vi "Logging.vi"(7 "CSM Name":string="CSM-Module") -> ()   [LabVIEW 2026, in "UI-无创.lvlib" / "Logging.lvlib"]
uses:
  Logging.lvlib
  Supports/Logging States.ctl
  Supports/Sample Settings.ctl
  Supports/Time and Data_OP.ctl
  4d3beaf1-401a-43cb-9e41-e4ff7a78e202.vi
  1a146c5b-3d51-4d3e-9388-f96b0b9a5a8e.vi
  <userlib>/_NEVSTOP/Communicable State Machine(CSM)/AdvanceAPI/CSM - Revert Arguments-Safe String.vi
  <userlib>/_NEVSTOP/Communicable State Machine(CSM)/_Shared/Trim Single-line Text.vi
  <userlib>/_NEVSTOP/Communicable State Machine(CSM)/AdvanceAPI/CSM - Make String Arguments Safe.vi
  <userlib>/_NEVSTOP/Communicable State Machine(CSM)/AdvanceAPI/CSM - Break Down Multiple States String.vi
  <userlib>/_NEVSTOP/Communicable State Machine(CSM)/AdvanceAPI/CSM - Compact Multiple States.vi
  <userlib>/_NEVSTOP/Communicable State Machine(CSM)/AdvanceAPI/CSM - Keywords.vi
  <userlib>/_NEVSTOP/Communicable State Machine(CSM)/addons/API-String-Arugments-Support/_Support/Convert API String Arguments to Data(variant).vi
  <userlib>/_NEVSTOP/Communicable State Machine(CSM)/addons/MassData-Parameter/_support/FGV-MassData(lvlibp).vi
  <userlib>/_NEVSTOP/Communicable State Machine(CSM)/Communicable State Machine.lvlib
panel:
  out "Error Occurred":errorcluster
  out "State History":string
  in  "Exit":bool
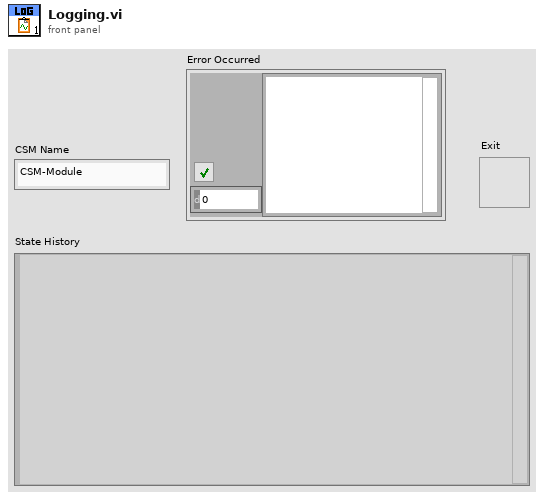
[diagram p1: front panel]
types:
  T1 = enum32{"Invalid", "Standard", "Closed", "Hidden", "Minimized", "Maximized"}
  T2 = enum32{"invalid app kind", "Development System", "Run Time System", "Student Edition", "Embedded LabVIEW", "Evaluation", "Custom"}
  T3 = typedef "UI-无创.lvlib/Logging.lvlib/Logging States.ctl" = enum16{"Idle", "Logging", "Error"}
  T4 = typedef "Communicable State Machine.lvlib/_CSM_Response Source Message.ctl" = cluster{"‘State":string, "’Arguments":string, "’Error":errorcluster}
  T5 = cluster{"Current VI Reference":refnum<vi>, "Close Panel on Exit?":bool}
  T6 = typedef "UI-无创.lvlib/Sample Settings.ctl" = cluster{"设备信息":cluster{"初始索引子集":i8[], "模拟信号采集通道":string, "数字-供电":refnum<k21>, "数字-光控":refnum<k21>, "光控设备":tag, "光电设备分离？":bool, "光谱保存路径":path, "环数":u8}, "测量控制":cluster{"测头拿起":bool, "起始保存":bool, "测头供电":bool, "测头出光":bool}, "测量":cluster{"每波长测量次数":i32, "波长":i32[], "起始周期":i32, "起始测量周期":i32}, "等待":cluster{"等待时间(s)":dbl, "等待方式":bool, "每x周期/点等待":i32, "等待时":enum16{"无电无光", "有电无光", "无电有光", "有电有光"}}, "校准":cluster{"暗电流校准值初值":dbl[], "温度校准值":dbl[], "校准模式":T7}, "图表相关":cluster{"文件-时间":string}, "CSM":cluster{"CSM Name":string}}
  T7 = typedef "UI-无创.lvlib/暗电流校准模式.ctl" = enum32{"手动", "逐周期"}
  T8 = cluster{"Core":cluster{"Current VI Reference":refnum<vi>, "Close Panel on Exit?":bool}, "Logging State":T3, "Sample Settings":T6}
  T9 = typedef "UI-无创.lvlib/Time and Data_OP.ctl" = cluster{"采集时间":timestamp, "采集时间(dbl)":dbl, "Data":dbl[], "当前运行信息":cluster{"当前周期":i32, "当前次数":i32, "测量周期":i32, "当前索引子集":i8[], "当前波长":i32}, "暗电流校准值":dbl[], "Logging Settings":cluster{"是否保存？":bool, "波长结束？":bool, "周期结束？":bool}, "原始值":cluster{"1环(原始值)":dbl[][], "2环(原始值)":dbl[][], "3环(原始值)":dbl[][], "4环(原始值)":dbl[][], "5环(原始值)":dbl[][], "6环(原始值)":dbl[][], "7环(原始值)":dbl[][]}, "校准值":cluster{"1环(校准值)":dbl[][], "2环(校准值)":dbl[][], "3环(校准值)":dbl[][], "4环(校准值)":dbl[][], "5环(校准值)":dbl[][], "6环(校准值)":dbl[][], "7环(校准值)":dbl[][]}}
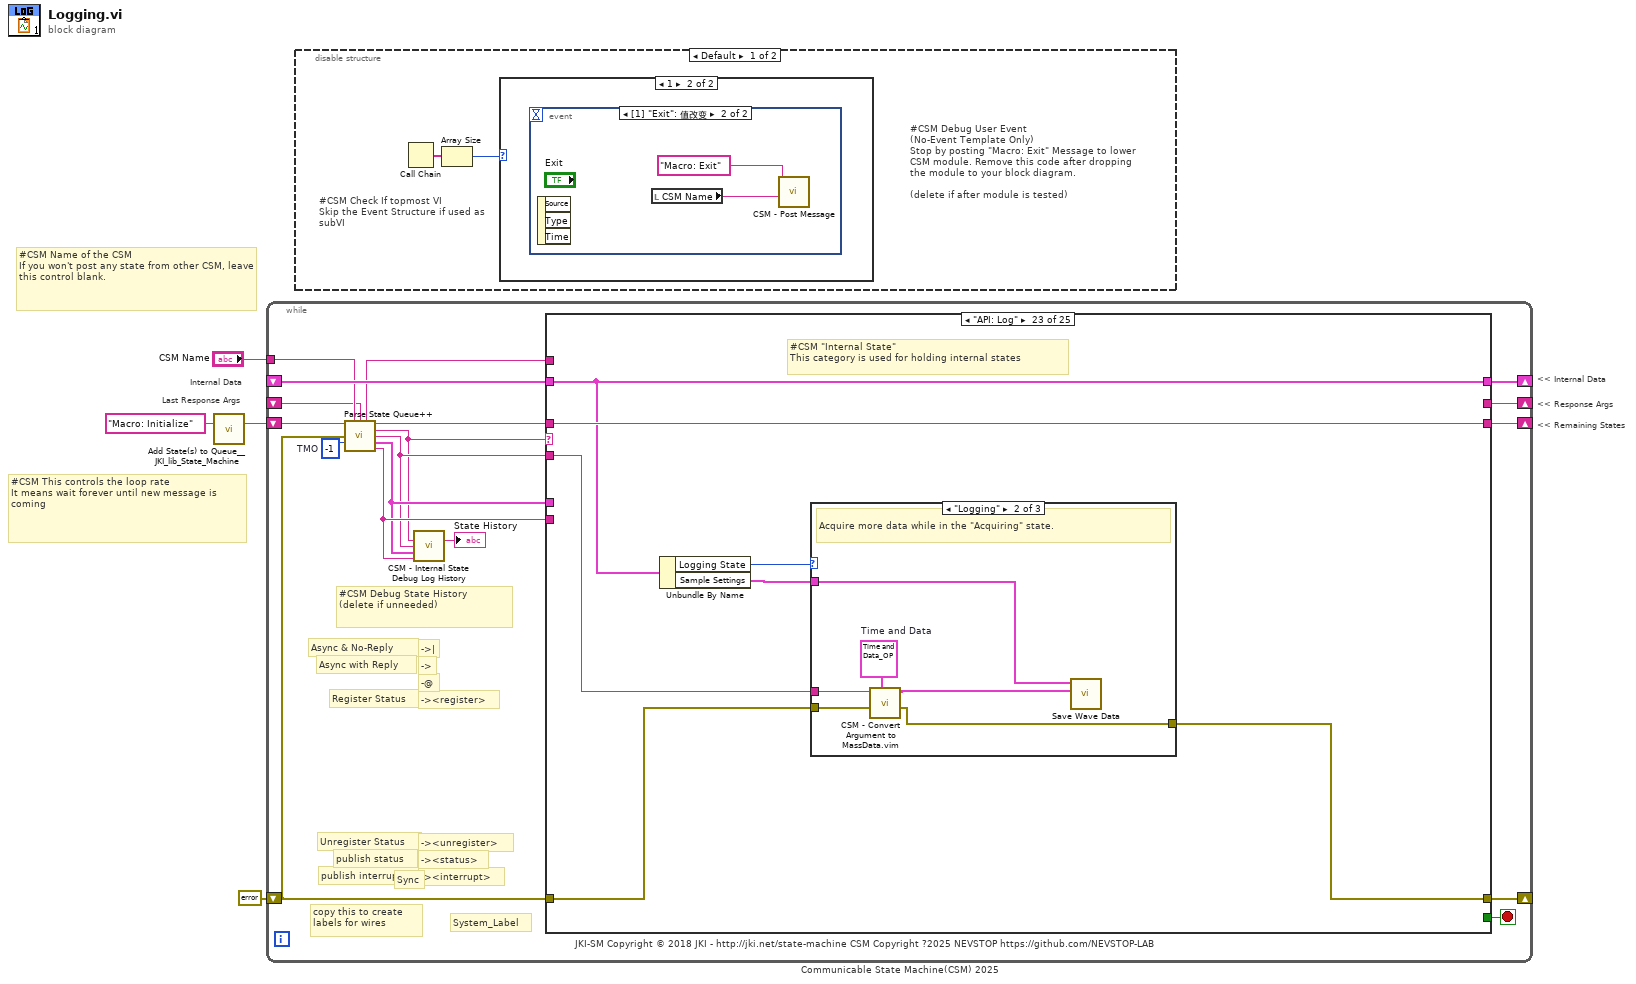
[diagram p0: block diagram]
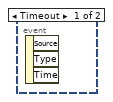
[diagram p3: hidden frame]
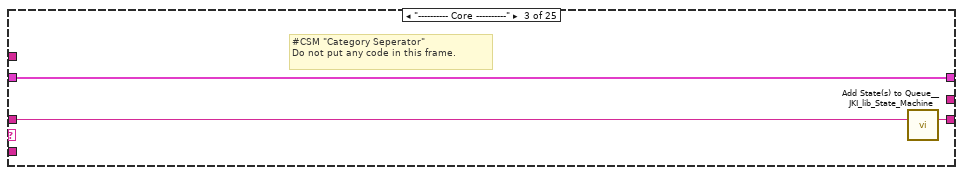
[diagram p7: hidden frame]
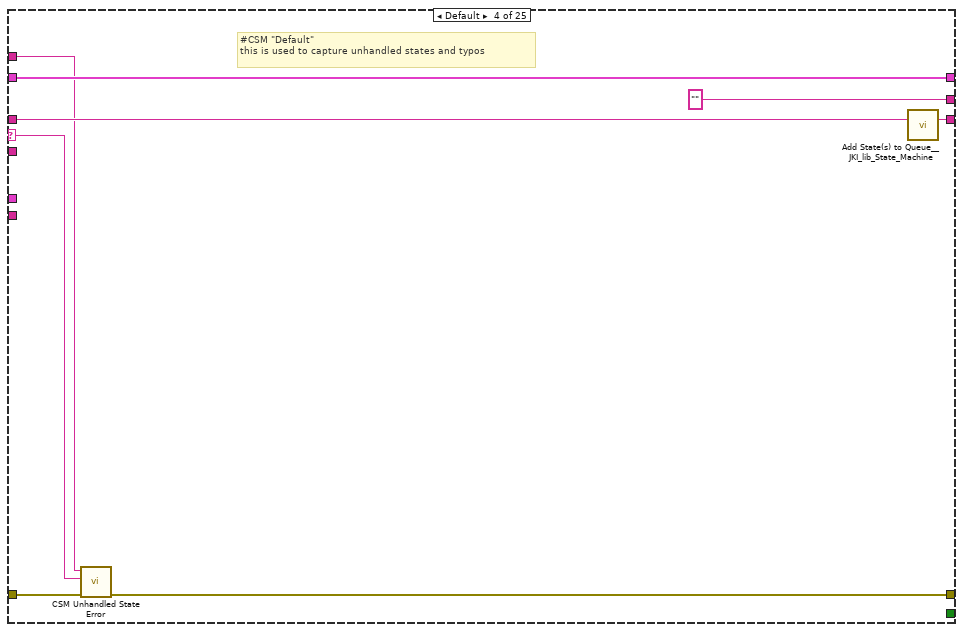
[diagram p8: hidden frame]
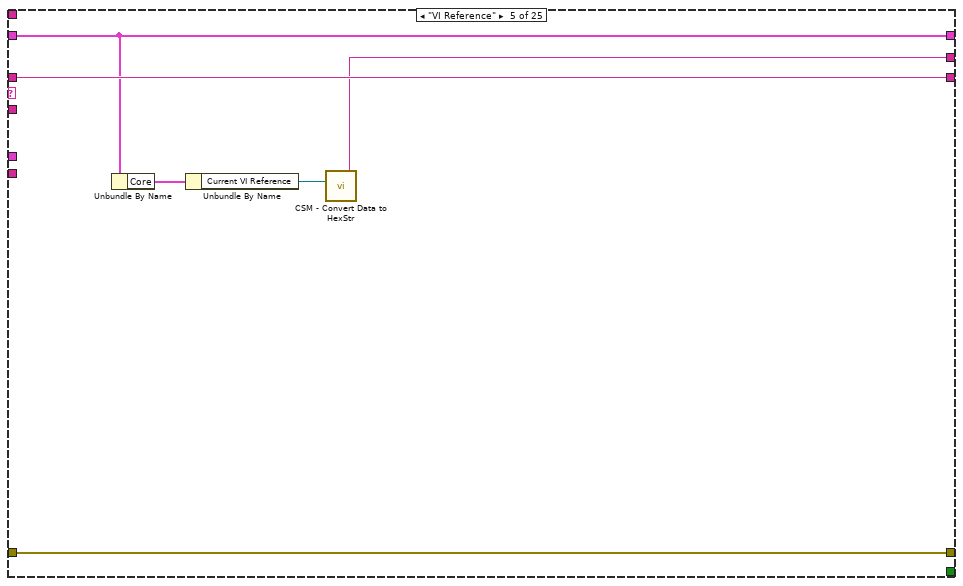
[diagram p9: hidden frame]
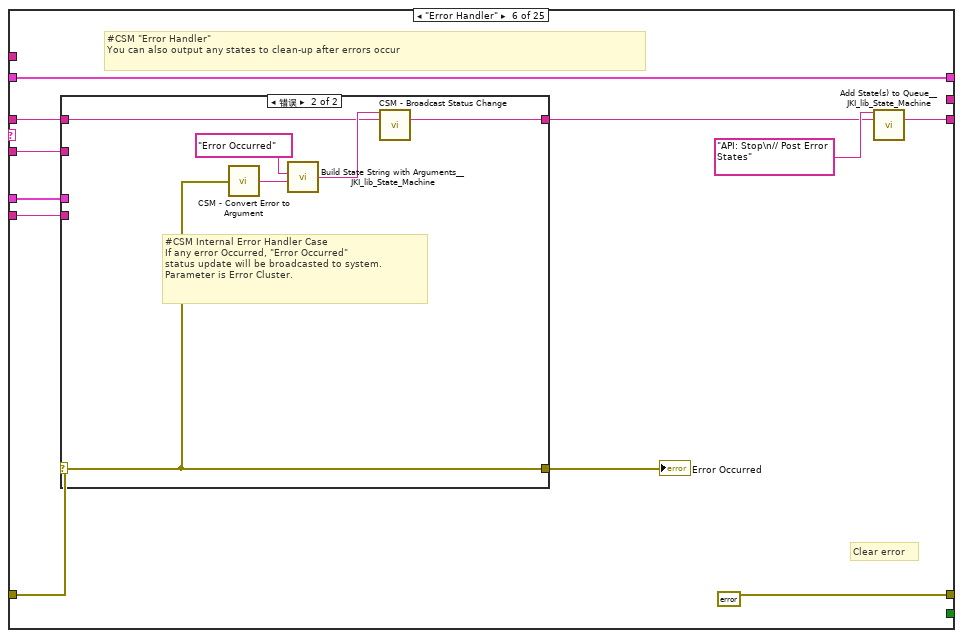
[diagram p10: hidden frame]
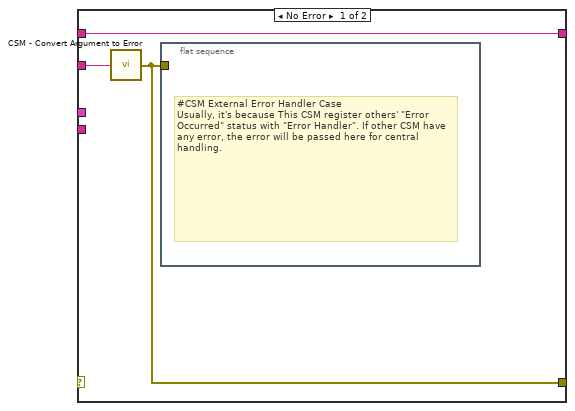
[diagram p11: hidden frame]
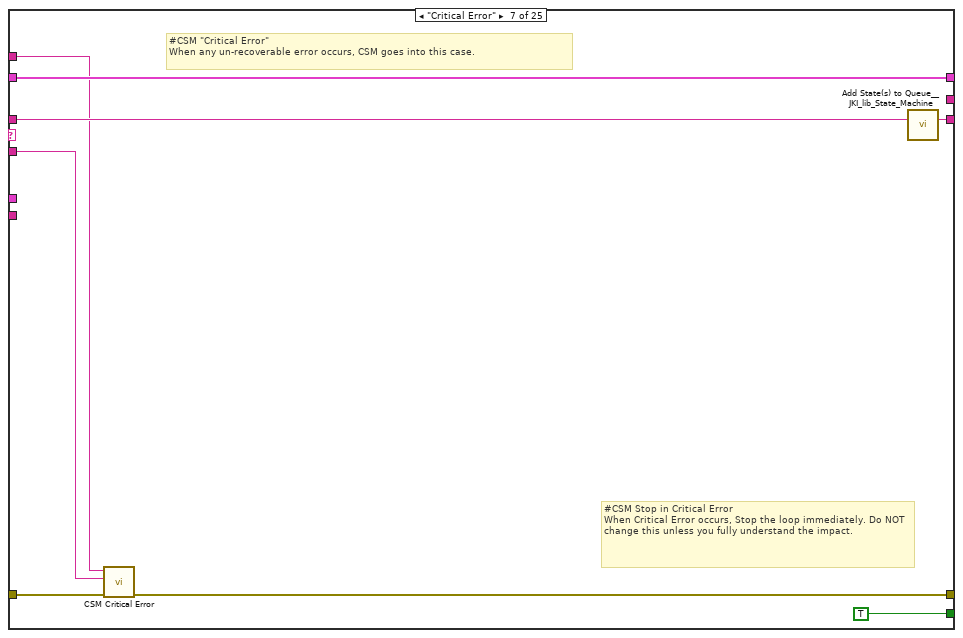
[diagram p12: hidden frame]
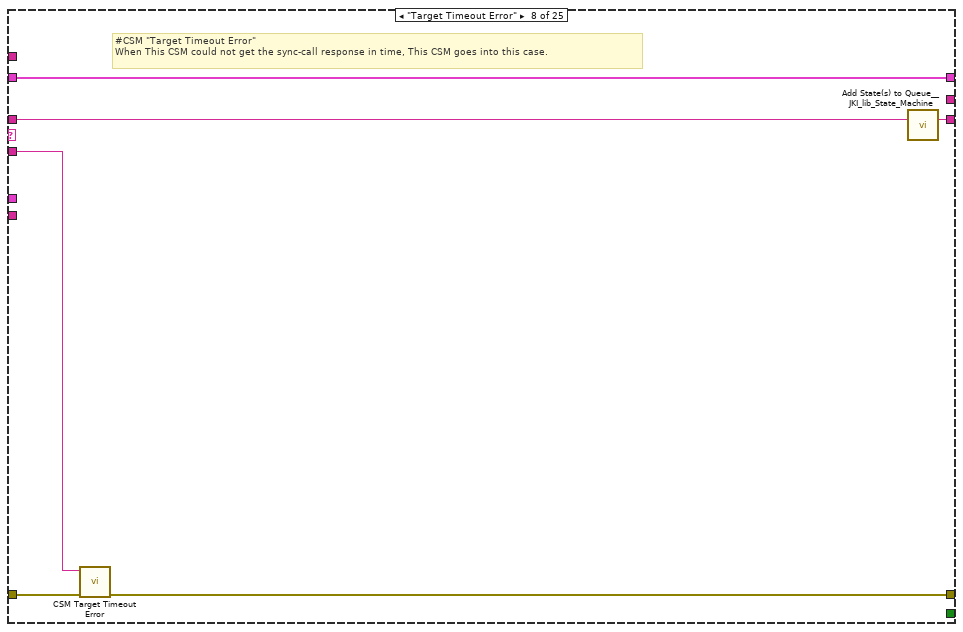
[diagram p13: hidden frame]
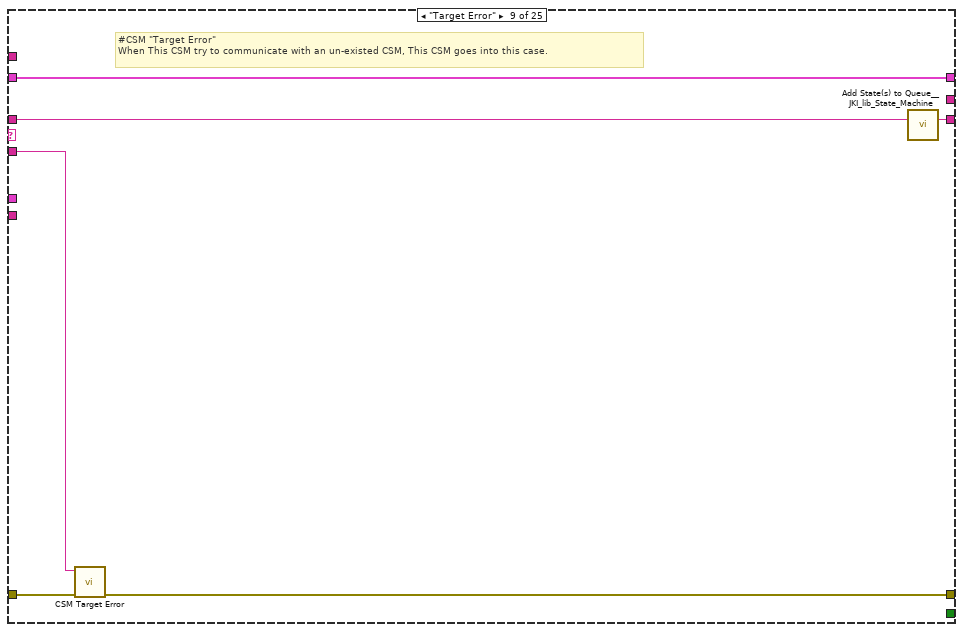
[diagram p14: hidden frame]
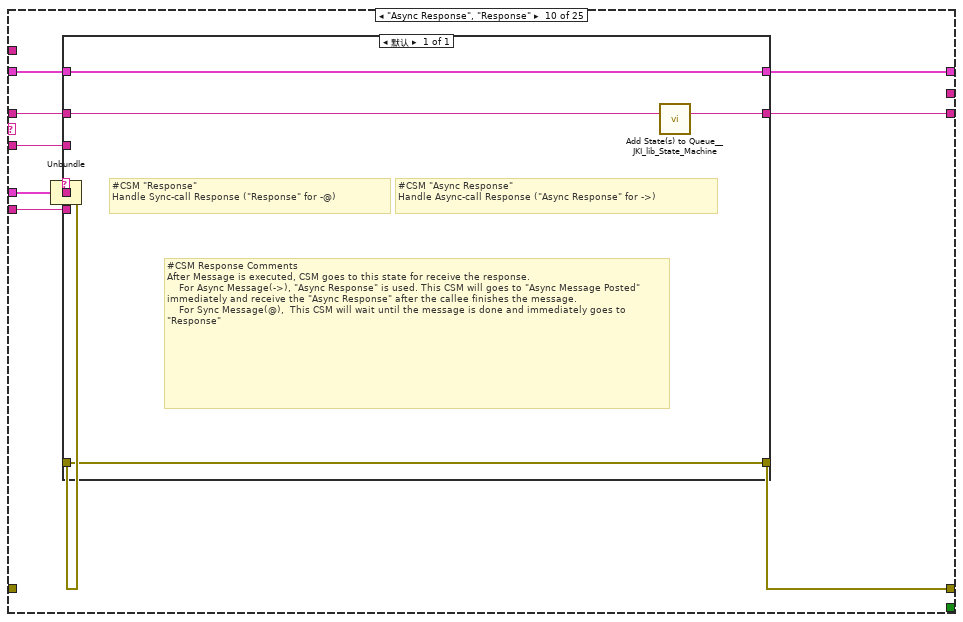
[diagram p15: hidden frame]
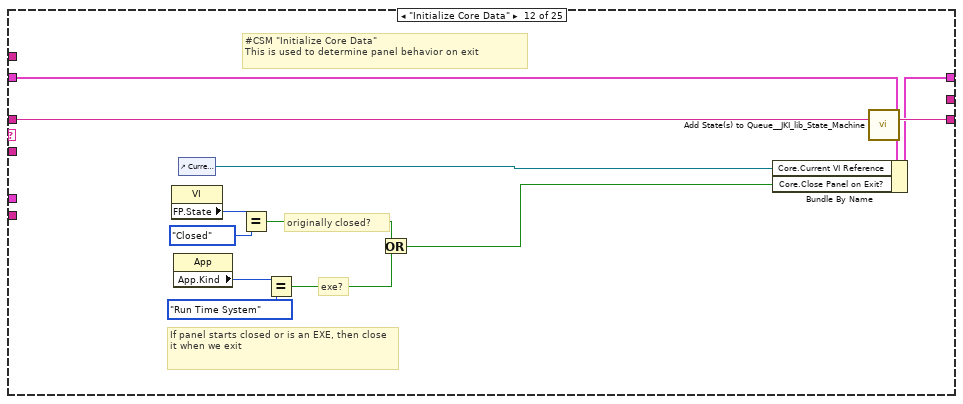
[diagram p17: hidden frame]
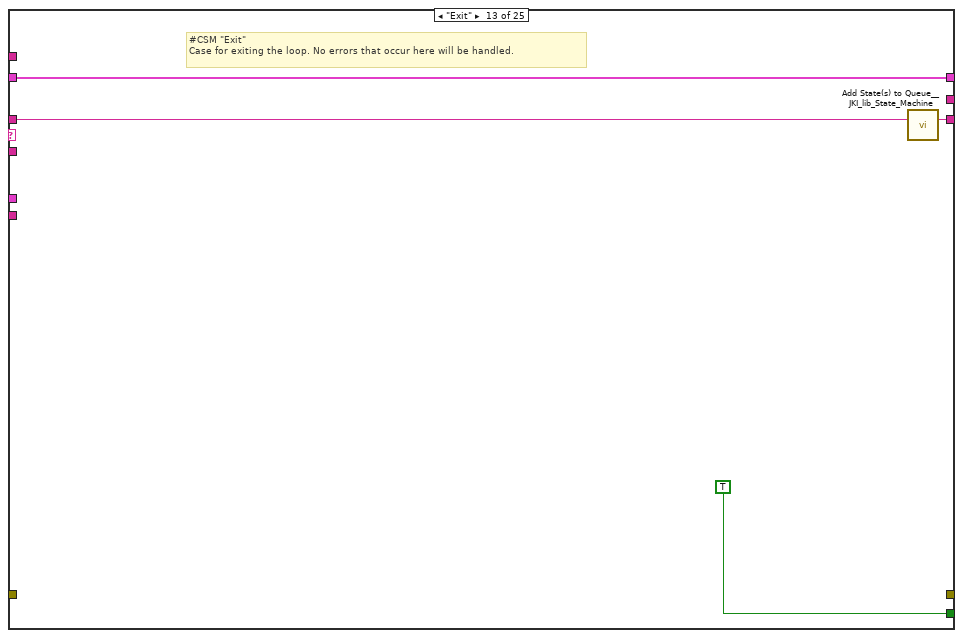
[diagram p18: hidden frame]
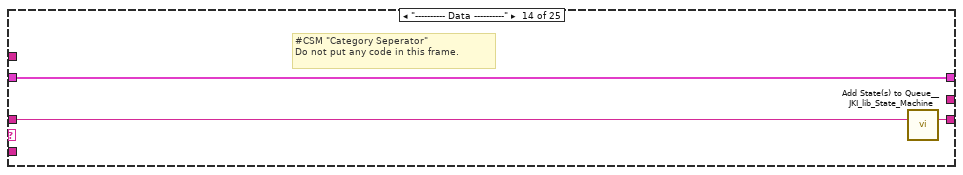
[diagram p19: hidden frame]
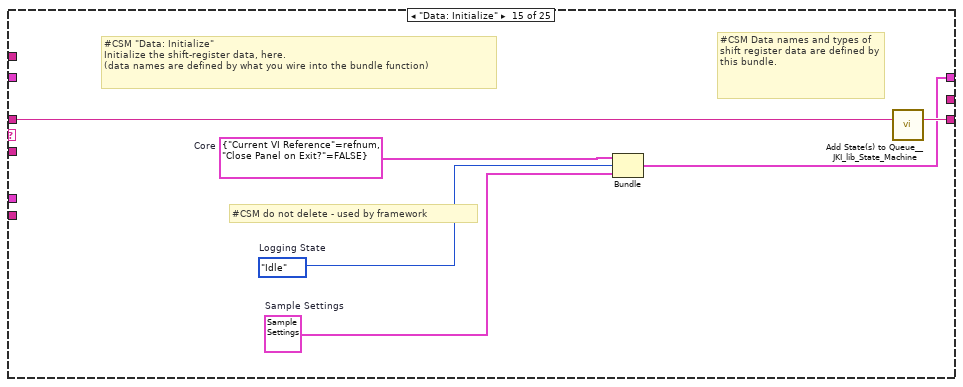
[diagram p20: hidden frame]
diagram:
  # "Last Response Args"
  # "Internal Data"
  # "#CSM Name of the CSM\nIf you won't post any state from other CSM, leave this control blank."
  # "#CSM This controls the loop rate\nIt means wait forever until new message is coming"
  # "<< Internal Data"
  # "<< Response Args"
  # "<< Remaining States"
  n1 = call <vilib>:"Add State(s) to Queue__JKI_lib_State_Machine.vi"("State(s) in (\"\")"="Macro: Initialize" ("Init State(\"Macro: Initialize\")")) -> ("States Out"=w1:string)  [unwired: 14 in]
  n2 = while "Communicable State Machine(CSM) 2025" {
    shift-right: [w17] -> _
    shift-left: _ -> [w16]
    shift-right: [w20] -> _
    shift-left: errorcluster {"status"=FALSE, "code"=0, "source"=""} ("error out") -> [w6]
    shift-right: [w19] -> _
    shift-left: w1 -> [w21]
    tunnel: "CSM Name" -> [w13]
    shift-right: [w14] -> _
    shift-left: _ -> [w8]
    stop <- w18 stop-if-true
    w15 = -1  # TMO
    # "#CSM Debug State History\n(delete if unneeded)"
    # "-><interrupt>"
    # "-><status>"
    # "-><unregister>"
    # "-><register>"
    # "-@"
    # "->"
    # "->|"
    # "publish interrupt"
    # "publish status"
    # "Unregister Status"
    # "Register Status"
    # "Sync"
    # "Async with Reply"
    # "Async & No-Reply"
    # "JKI-SM Copyright © 2018 JKI - http://jki.net/state-machine CSM Copyright ?2025 NEVSTOP https://github.com/NEVSTOP-LAB"
    # "copy this to create labels for wires"
    # "System_Label"
    n3 = call <userlib>:"Parse State Queue++.vi"("State Queue"=w21, "Name (\"\" to Use UUID)"=w13, "Response Arguments"=w8, "Previous Error"=w6, "Dequeue (1 ms)"=w15) -> ("Name Used"=w7:string, "Remaining States"=w22:string, "Current State"=w9:string, "Arguments"=w10:string, "Additional Information"=w11:T4, "Source CSM"=w12:string)  [unwired: 5 in]
    n4 = call <userlib>:"CSM - Internal State Debug Log History.vi"("State"=w9, "Arguments (\"\")"=w10, ">> Response Source Message >>"=w11, "Source (\"\")"=w12) -> ("Debug Log"=→"State History":string)  [unwired: 11 in]
    n5 = case shown="\"API: Log\"" w9 {
      selector: w9 -> [_ _ _ w33 _ _ _ _ _ _ _ _ _ _ _ _ _ _ _ _ _ _ _ _ _]
      tunnel: w22 -> [w23 w26 w29 w37 w42 w48 w71 w77 w83 w93 w100 w112 w116 w119 w125 w128 w134 w137 w141 w147 w149 w156 w170 w184 w193]
      tunnel: w10 -> [_ _ _ _ _ w47 w67 w74 w80 w87 _ _ _ _ _ _ _ _ _ _ _ w151 w168 _ _]
      tunnel: w16 -> [w24 w25 w27 w35 w41 w53 w69 w75 w81 w91 w99 w106 w114 w117 _ w127 w129 w135 w139 w145 w150 w155 w169 w185 w191]
      tunnel: [_ _ _ w30 w43 errorcluster {"status"=FALSE, "code"=0, "source"=""} ("error out") w64 w72 w78 w94 _ _ _ _ _ _ w130 _ _ _ _ w152 w171 _ _] -> w20
      tunnel: w6 -> [_ _ _ w31 w43 w51 w65 w73 w79 _ _ _ _ _ _ _ w131 _ _ _ _ w152 w172 _ _]
      tunnel: [w23 w26 w28 w36 w42 w49 w70 w76 w82 w92 w100 w111 w115 w118 w124 w128 w133 w136 w140 w146 w148 w156 w170 w183 w192] -> w19
      tunnel: [_ _ _ _ _ _ TRUE _ _ _ _ _ TRUE _ _ _ _ _ _ _ _ _ _ _ _] -> w18
      tunnel: [w24 w25 w27 w35 w41 w53 w69 w75 w81 w90 w99 w110 w114 w117 w123 w127 w129 w135 w139 w145 w150 w154 w169 w185 w190] -> w17
      tunnel: w12 -> [_ _ _ _ _ w46 _ _ _ w88 _ _ _ _ _ _ _ _ _ _ _ _ _ _ _]
      tunnel: w11 -> [_ _ _ _ _ w45 _ _ _ w89 _ _ _ _ _ _ _ _ _ _ _ _ _ _ _]
      tunnel: [_ _ _ "" w38 _ _ _ _ _ _ _ _ _ _ _ _ _ _ _ _ _ _ _ _] -> w14
      tunnel: w7 -> [_ _ _ w32 _ _ w66 _ _ _ _ _ _ _ _ _ _ _ _ _ _ w153 _ _ _]
      frame "", "Idle" {
        # "#CSM \"Idle/Event Handler\"\nexecutes when the state queue is empty"
      }
      frame "CSM Documentation" {
        # "#CSM State Syntax\n\n// Comment line, all text to the right of “//” will be ignored\n// Local Message Example\nDoSth: DoA >> Arguments\n\n// Sync Call Example\nAPI: xxxx >> Arguments -@ TargetModule\n\n// Async Call Example\nAPI: xxxx >> Arguments -> TargetModule\n\n// Async Call without Reply Example\nAPI: xxxx >> Arguments ->| TargetModule\n\n// Broadcast normal status:\nStatus >> StatusArguments  -><status>\n\n// Broadcast Interrupt status:\nInterrupt >> StatusArguments  -><interrupt>\n\n// Register Source Module's status to Handler Module\nStatus@Source Module >> Handler Module@Handler Module -><register>\n\n// Unegister Source Module's status\nStatus@Source Module >> Handler Module -><unregister>"
        # "#CSM README FIRST\n\nCommunicable State Machine(CSM) is a LabVIEW application framework that builds upon JKI State Machine(JKISM). It follows the pattern of JKISM and extends the keywords to describe message communication between modules, including concepts such as Sync-Message, Async-Message, Subscription/Unsubscription of status - essential elements for creating reusable code modules. For more information, please visit the CSM wiki: https://nevstop-lab.github.io/CSM-Wiki/\n\nFor instructions on JKI State Machine, visit: \n    http://jki.net/state-machine/\nFor information about CSM, visit: \n    https://github.com/NEVSTOP-LAB"
        # "#CSM \"Documentation\"\nCase for holding CSM Documenation"
      }
      frame "---------- Core ----------" {
        # "#CSM \"Category Seperator\"\nDo not put any code in this frame."
        n6 = call <vilib>:"Add State(s) to Queue__JKI_lib_State_Machine.vi"("State(s) in (\"\")"=w29) -> ("States Out"=w28:string)  [unwired: 14 in]
      }
      frame Default {
        # "#CSM \"Default\"\nthis is used to capture unhandled states and typos"
        n7 = call <userlib>:"CSM Unhandled State Error.vi"("error in (no error)"=w31, "Undefined State"=w33, "CSM Name"=w32) -> ("error out"=w30:errorcluster)  [unwired: 8 in]
        n8 = call <vilib>:"Add State(s) to Queue__JKI_lib_State_Machine.vi"("State(s) in (\"\")"=w37) -> ("States Out"=w36:string)  [unwired: 14 in]
      }
      frame "VI Reference" {
        n9 = Unbundle By Name(w41) -> ("Core"=w40:T5)
        n10 = Unbundle By Name(w40) -> ("Current VI Reference"=w39:refnum<vi>)
        n11 = call <userlib>:"CSM - Convert Data to HexStr.vi"("Variant"=w39) -> ("HEX String (0-9,A-F)"=w38:string)  [unwired: 8 in]
      }
      frame "Error Handler" {
        # "#CSM \"Error Handler\"\nYou can also output any states to clean-up after errors occur"
        # "Clear error"
        n12 = case shown="错误" w51 {
          selector: w51 -> [_ w58]
          tunnel: [w57 w60] -> w50
          tunnel: w48 -> [w57 w59]
          tunnel: w47 -> [w56 _]
          tunnel: w46 -> [_ _]
          tunnel: w45 -> [_ _]
          tunnel: [w55 w58] -> w44
          frame No Error {
            n13 = call <userlib>:"CSM - Convert Argument to Error.vi"("Argument"=w56) -> ("Error"=w55:errorcluster)  [unwired: 4 in]
            n14 = flat-sequence {
              tunnel: w55 -> [_]
              frame #0 {
                # "#CSM External Error Handler Case\nUsually, it's because This CSM register others' \"Error Occurred\" status with \"Error Handler\". If other CSM have any error, the error will be passed here for central handling."
              }
            }
          }
          frame Error {
            # "#CSM Internal Error Handler Case \nIf any error Occurred, \"Error Occurred\" \nstatus update will be broadcasted to system.\nParameter is Error Cluster."
            n15 = call <userlib>:"CSM - Convert Error to Argument.vi"("Error"=w58) -> ("Argument"=w62:string)  [unwired: 4 in]
            n16 = call <vilib>:"Build State String with Arguments__JKI_lib_State_Machine.vi"("Arguments (\"\")"=w62, "State"="Error Occurred" ("Status with Arguments")) -> ("State with Arguments"=w61:string)  [unwired: 4 in]
            n17 = call <userlib>:"CSM - Broadcast Status Change.vi"("Status With Arguments"=w61, "State Queue"=w59) -> ("Remaining States"=w60:string)  [unwired: 13 in]
          }
        }
        "Error Occurred" <- w44
        n18 = call <vilib>:"Add State(s) to Queue__JKI_lib_State_Machine.vi"("State(s) in Front (\"\")"="API: Stop\n// Post Error States", "State(s) in (\"\")"=w50) -> ("States Out"=w49:string)  [unwired: 13 in]
      }
      frame "Critical Error" {
        # "#CSM \"Critical Error\"\nWhen any un-recoverable error occurs, CSM goes into this case."
        # "#CSM Stop in Critical Error\nWhen Critical Error occurs, Stop the loop immediately. Do NOT change this unless you fully understand the impact."
        n19 = call <userlib>:"CSM Critical Error.vi"("error in (no error)"=w65, "Arugments (As Reason)"=w67, "CSM Name"=w66) -> ("error out"=w64:errorcluster)  [unwired: 8 in]
        n20 = call <vilib>:"Add State(s) to Queue__JKI_lib_State_Machine.vi"("State(s) in (\"\")"=w71) -> ("States Out"=w70:string)  [unwired: 14 in]
      }
      frame "Target Timeout Error" {
        # "#CSM \"Target Timeout Error\"\nWhen This CSM could not get the sync-call response in time, This CSM goes into this case."
        n21 = call <userlib>:"CSM Target Timeout Error.vi"("error in (no error)"=w73, "Arguments (As CSM Name)"=w74) -> ("error out"=w72:errorcluster)  [unwired: 9 in]
        n22 = call <vilib>:"Add State(s) to Queue__JKI_lib_State_Machine.vi"("State(s) in (\"\")"=w77) -> ("States Out"=w76:string)  [unwired: 14 in]
      }
      frame "Target Error" {
        # "#CSM \"Target Error\"\nWhen This CSM try to communicate with an un-existed CSM, This CSM goes into this case."
        n23 = call <userlib>:"CSM Target Error.vi"("error in (no error)"=w79, "Arguments (As CSM Name)"=w80) -> ("error out"=w78:errorcluster)  [unwired: 9 in]
        n24 = call <vilib>:"Add State(s) to Queue__JKI_lib_State_Machine.vi"("State(s) in (\"\")"=w83) -> ("States Out"=w82:string)  [unwired: 14 in]
      }
      frame "Async Response", "Response" {
        n25 = Unbundle(w89) -> ("‘State"=w86:string, "’Arguments"=w85:string, "’Error"=w84:errorcluster)
        n26 = case shown="默认" w86 {
          tunnel: [w95] -> w92
          tunnel: w93 -> [w96]
          tunnel: [w98] -> w90
          tunnel: w91 -> [w98]
          tunnel: [w97] -> w94
          tunnel: w84 -> [w97]
          tunnel: w88 -> [_]
          tunnel: w87 -> [_]
          tunnel: w85 -> [_]
          frame 默认 {
            # "#CSM \"Async Response\"\nHandle Async-call Response (\"Async Response\" for ->)"
            # "#CSM \"Response\"\nHandle Sync-call Response (\"Response\" for -@)"
            # "#CSM Response Comments\nAfter Message is executed, CSM goes to this state for receive the response.\n    For Async Message(->), \"Async Response\" is used. This CSM will goes to \"Async Message Posted\" immediately and receive the \"Async Response\" after the callee finishes the message.\n    For Sync Message(@),  This CSM will wait until the message is done and immediately goes to \"Response\""
            n27 = call <vilib>:"Add State(s) to Queue__JKI_lib_State_Machine.vi"("State(s) in (\"\")"=w96) -> ("States Out"=w95:string)  [unwired: 14 in]
          }
        }
      }
      frame "Async Message Posted" {
        # "#CSM \"Async Message Posted\"\nAfter Async Message is posted (-> or ->| ), CSM goes to this state for post-action.\nYou can use Argument - State to tell which Async Message is called."
      }
      frame "Initialize Core Data" {
        # "#CSM \"Initialize Core Data\"\nThis is used to determine panel behavior on exit"
        # "originally closed?"
        # "exe?"
        # "If panel starts closed or is an EXE, then close it when we exit"
        n28 = property class="VI"() -> ("FP.State"=w103:T1)  [unwired: 2 in, 2 out]
        n29 = property class="App"() -> ("App.Kind"=w109:T2)  [unwired: 2 in, 2 out]
        n30 = control-ref of="Current VI Reference"() -> (w104:refnum<vi>)
        n31 = Equal?(x=w103, y=T1."Closed" ("Front Panel Window:State")) -> (x = y?=w101:bool)
        n32 = Equal?(x=w109, y=T2."Run Time System" ("Application:Kind")) -> (x = y?=w107:bool)
        n33 = Or(x=w101, y=w107) -> (x .or. y?=w105:bool)
        n34 = Bundle By Name(cluster=w106, "Core.Current VI Reference"=w104, "Core.Close Panel on Exit?"=w105) -> (w110:T8)
        n35 = call <vilib>:"Add State(s) to Queue__JKI_lib_State_Machine.vi"("State(s) in (\"\")"=w112) -> ("States Out"=w111:string)  [unwired: 14 in]
      }
      frame "Exit" {
        # "#CSM \"Exit\"\nCase for exiting the loop. No errors that occur here will be handled."
        n36 = call <vilib>:"Add State(s) to Queue__JKI_lib_State_Machine.vi"("State(s) in (\"\")"=w116) -> ("States Out"=w115:string)  [unwired: 14 in]
      }
      frame "---------- Data ----------" {
        # "#CSM \"Category Seperator\"\nDo not put any code in this frame."
        n37 = call <vilib>:"Add State(s) to Queue__JKI_lib_State_Machine.vi"("State(s) in (\"\")"=w119) -> ("States Out"=w118:string)  [unwired: 14 in]
      }
      frame "Data: Initialize" {
        w120 = T6 {"设备信息"={"初始索引子集"=[], "模拟信号采集通道"="", "数字-供电"="", "数字-光控"="", "光控设备"="", "光电设备分离？"=FALSE, "光谱保存路径"=path "", "环数"=0}, "测量控制"={"测头拿起"=FALSE, "起始保存"=FALSE, "测头供电"=TRUE, "测头出光"=TRUE}, "测量"={"每波长测量次数"=5, "波长"=[0, 0, 0, 0, 0, 0], "起始周期"=0, "起始测量周期"=0}, "等待"={"等待时间(s)"=0.0, "等待方式"=FALSE, "每x周期/点等待"=8, "等待时"=enum."无电无光"}, "校准"={"暗电流校准值初值"=[], "温度校准值"=[0.0, 0.0, 0.0, 0.0, 0.0, 0.0, 0.00013, 0.00013, 0.00013, 0.00013, 0.00013, 0.00013], "校准模式"=enum."逐周期"}, "图表相关"={"文件-时间"=""}, "CSM"={"CSM Name"=""}}  # Sample Settings
        w121 = Logging_States."Idle"  # Logging State
        w122 = T5 {"Current VI Reference"=refnum, "Close Panel on Exit?"=FALSE}  # Core
        # "#CSM \"Data: Initialize\"\nInitialize the shift-register data, here.\n(data names are defined by what you wire into the bundle function)"
        # "#CSM do not delete - used by framework"
        # "#CSM Data names and types of shift register data are defined by this bundle."
        n38 = Bundle("Core"=w122, "Logging State"=w121, "Sample Settings"=w120) -> (w123:T8)  [unwired: 1 in]
        n39 = call <vilib>:"Add State(s) to Queue__JKI_lib_State_Machine.vi"("State(s) in (\"\")"=w125) -> ("States Out"=w124:string)  [unwired: 14 in]
      }
      frame "Data: Update Indicators" {
        n40 = local write "Error Occurred"(errorcluster {"status"=FALSE, "code"=0, "source"=""} ("错误常量")) -> ()
      }
      frame "Data: Cleanup" {
        # "#CSM \"Data: Cleanup\"\nCleanup any data and references, here.\n(this is called automatically, by the Macro: Exit)"
        n41 = Unbundle By Name(w129) -> ("Core.Current VI Reference"=w132:refnum<vi>)
        n42 = Close Reference(reference=w132, error in (no error)=w131) -> (error out=w130:errorcluster)
        n43 = call <vilib>:"Add State(s) to Queue__JKI_lib_State_Machine.vi"("State(s) in (\"\")"=w134) -> ("States Out"=w133:string)  [unwired: 14 in]
      }
      frame "---------- Macro ----------" {
        # "#CSM \"Category Seperator\"\nDo not put any code in this frame."
        n44 = call <vilib>:"Add State(s) to Queue__JKI_lib_State_Machine.vi"("State(s) in (\"\")"=w137) -> ("States Out"=w136:string)  [unwired: 14 in]
      }
      frame "Macro: Initialize" {
        # "#CSM \"Macro: Initialize\"\nInitialization Macro (This is called once, when the VI starts)"
        n45 = call <vilib>:"Add State(s) to Queue__JKI_lib_State_Machine.vi"("State(s) in Front (\"\")"="Data: Initialize\nInitialize Core Data\nData: Update Indicators", "State(s) in (\"\")"=w141) -> ("States Out"=w140:string)  [unwired: 13 in]
      }
      frame "Macro: Exit" {
        # "#CSM \"Macro: Exit\"\nExit Macro (This is called once, when the VI exits)"
        n46 = call <vilib>:"Add State(s) to Queue__JKI_lib_State_Machine.vi"("State(s) in Front (\"\")"="//Exit Sub-Modules ", "State(s) at Back (\"\")"="Data: Cleanup\nExit") -> ("States Out"=w143:string)  [unwired: 13 in]
        n47 = call <vilib>:"Add State(s) to Queue__JKI_lib_State_Machine.vi"("State(s) in Front (\"\")"=w143, "State(s) in (\"\")"=w147) -> ("States Out"=w146:string)  [unwired: 13 in]
      }
      frame "---------- API ----------" {
        # "#CSM \"Category Seperator\"\nDo not put any code in this frame."
        n48 = call <vilib>:"Add State(s) to Queue__JKI_lib_State_Machine.vi"("State(s) in (\"\")"=w149) -> ("States Out"=w148:string)  [unwired: 14 in]
      }
      frame "API: Start" {
        # "#CSM API Example\nCopy/Rename this case for your own API"
        n49 = Unbundle By Name(w155) -> ("Logging State"=w158:T3)
        n50 = case shown="\"Idle\", 默认" w158 {
          tunnel: w155 -> [w164 w165 w166]
          tunnel: [w163 w165 w166] -> w154
          tunnel: w153 -> [_ _ _]
          tunnel: w151 -> [w161 _ _]
          frame "Idle", Default {
            w160 = T6 {"设备信息"={"初始索引子集"=[], "模拟信号采集通道"="", "数字-供电"="", "数字-光控"="", "光控设备"="", "光电设备分离？"=FALSE, "光谱保存路径"=path "", "环数"=0}, "测量控制"={"测头拿起"=FALSE, "起始保存"=FALSE, "测头供电"=TRUE, "测头出光"=TRUE}, "测量"={"每波长测量次数"=5, "波长"=[0, 0, 0, 0, 0, 0], "起始周期"=0, "起始测量周期"=0}, "等待"={"等待时间(s)"=0.0, "等待方式"=FALSE, "每x周期/点等待"=8, "等待时"=enum."无电无光"}, "校准"={"暗电流校准值初值"=[], "温度校准值"=[0.0, 0.0, 0.0, 0.0, 0.0, 0.0, 0.00013, 0.00013, 0.00013, 0.00013, 0.00013, 0.00013], "校准模式"=enum."逐周期"}, "图表相关"={"文件-时间"=""}, "CSM"={"CSM Name"=""}}  # Sample Settings
            # "If the system is idle, start the acquisition."
            n51 = call "Convert API String Arguments to Data.vim"("Reference Type"=w160, "API String"=w161) -> ("Data"=w159:T6)  [unwired: 6 in, 1 out]
            n52 = Bundle By Name(cluster=w164, "Logging State"=Logging_States."Logging", "Sample Settings"=w159) -> (w163:T8)
          }
          frame "Logging" {
            # "The system is already acquiring. Ignore the \"Start\" message."
          }
          frame "Error" {
          }
        }
        n53 = local write "Error Occurred"(errorcluster {"status"=FALSE, "code"=0, "source"=""} ("错误常量")) -> ()
      }
      frame "API: Log" {
        # "#CSM \"Internal State\"\nThis category is used for holding internal states"
        n54 = Unbundle By Name(w169) -> ("Logging State"=w173:T3, "Sample Settings"=w167:T6)
        n55 = case shown="\"Logging\"" w173 {
          tunnel: [w174 w177 w181] -> w171
          tunnel: w172 -> [w174 w179 w181]
          tunnel: w168 -> [_ w180 _]
          tunnel: w167 -> [_ w176 _]
          frame "Idle" {
            # "Ignore \"Acquire\" messages when the acquisition is idle."
          }
          frame "Logging" {
            w178 = T9 {"采集时间"=timestamp(0 s since 1904-01-01), "采集时间(dbl)"=0.0, "Data"=[], "当前运行信息"={"当前周期"=0, "当前次数"=0, "测量周期"=0, "当前索引子集"=[], "当前波长"=0}, "暗电流校准值"=[], "Logging Settings"={"是否保存？"=FALSE, "波长结束？"=FALSE, "周期结束？"=FALSE}, "原始值"={"1环(原始值)"=[], "2环(原始值)"=[], "3环(原始值)"=[], "4环(原始值)"=[], "5环(原始值)"=[], "6环(原始值)"=[], "7环(原始值)"=[]}, "校准值"={"1环(校准值)"=[], "2环(校准值)"=[], "3环(校准值)"=[], "4环(校准值)"=[], "5环(校准值)"=[], "6环(校准值)"=[], "7环(校准值)"=[]}}  # Time and Data
            # "Acquire more data while in the \"Acquiring\" state."
            n56 = call "CSM - Convert Argument to MassData.vim"("Type"=w178, "error in (no error)"=w179, "MassData Argument"=w180) -> ("error out"=w177:errorcluster, "Data"=w175:T9)  [unwired: 5 in]
            n57 = call "Save Wave Data.vi"("Time and Data"=w175, "Sample Settings"=w176) -> ()  [unwired: 10 in]
          }
          frame "Error" {
          }
        }
      }
      frame "API: Stop" {
        # "#CSM API Example\nCopy/Rename this case for your own API"
        n58 = Unbundle By Name(w185) -> ("Logging State"=w186:T3)
        n59 = case shown="\"Logging\"" w186 {
          tunnel: [_ "API: Close" ("State(s) in Front (\"\")") "API: Close" ("State(s) in Front (\"\")")] -> w182
          frame "Idle" {
            # "The system is already idle. Ignore the \"Stop\" message."
          }
          frame "Logging" {
            # "If the system is acquiring, stop the acquisition."
          }
          frame "Error" {
          }
        }
        n60 = call <vilib>:"Add State(s) to Queue__JKI_lib_State_Machine.vi"("State(s) in Front (\"\")"=w182, "State(s) in (\"\")"=w184) -> ("States Out"=w183:string)  [unwired: 13 in]
      }
      frame "API: Close" {
        # "#CSM \"Internal State\"\nThis category is used for holding internal states"
        n61 = Bundle By Name(cluster=w191, "Logging State"=Logging_States."Idle") -> (w190:T8)
        n62 = call <vilib>:"Add State(s) to Queue__JKI_lib_State_Machine.vi"("State(s) in (\"\")"=w193) -> ("States Out"=w192:string)  [unwired: 14 in]
      }
    }
  }
  n63 = disable-structure shown="Default" {
    frame condition #0 (active) {
      # "#CSM Check If topmost VI\nSkip the Event Structure if used as subVI"
      # "#CSM Debug User Event\n(No-Event Template Only)\nStop by posting \"Macro: Exit\" Message to lower CSM module. Remove this code after dropping the module to your block diagram. \n\n(delete if after module is tested)"
      n64 = Call Chain() -> (call chain=w195:string[])
      n65 = Array Size(array=w195) -> (size(s)=w194:i32)
      n66 = case shown="1" w194 {
        frame Default {
        }
        frame 1 {
          n67 = event shown="[1] \"Exit\": 值改变" {
            selector: _ -> [_ _]
            dyn-events: _ -> [_ _]
            timeout: _ -> [_ _]
            event Timeout {
              n68 = event-data() -> ()  [unwired: 1 in, 3 out]
            }
            event "Exit": Value Change {
              n69 = event-data() -> ()  [unwired: 1 in, 3 out]
              n70 = local read "CSM Name"() -> (w197:string)
              n71 = call <userlib>:"CSM - Post Message.vi"("Target Module"=w197, "State"="Macro: Exit" ("States")) -> ()  [unwired: 9 in, 1 out]
            }
          }
        }
      }
    }
    frame condition #1 {
    }
  }
